vi "VHistory - Control Center.vi"(4 "value condition":T2 {"Range_Max" format="%<%H:%M:%S%2u>t"; "Range_Min" format="%<%H:%M:%S%2u>t"; "Delta" format="%<%H:%M:%S%2u>t"}, 6 "time conditions":cluster{"Step, ms":u32, "Gate, ms":u32}, 7 "VC Handle":T4=-1, 8 "error in":errorcluster, 9 "cmd (nop:default)":T3(ring), 10 "history length":i32, 11 "name_spec":string) -> (0 "error out":errorcluster, 2 "history info":T1 {"last time, sec" format="%<%H:%M:%S%2u\n%d/%m/%Y>T"; "value condition"."Range_Max" format="%<%H:%M:%S%2u>t"; "value condition"."Range_Min" format="%<%H:%M:%S%2u>t"; "value condition"."Delta" format="%<%H:%M:%S%2u>t"}, 3 "dup name_spec":string)   [LabVIEW 2021]
doc: "The VI is obsolete. It only exists to provide compatibility with VarMan 2.1. Use 'VHistory - History Controller.vi' instead of this VI.\n\n::: CalcExpress Toolkit :::\nCopyright (c) 2000-2026 Konstantin Shifershteyn. All rights reserved."
uses:
  cetypes.llb/VarMan Variable Context Handle.ctl
panel:
  # "THIS VI IS OBSOLETE"
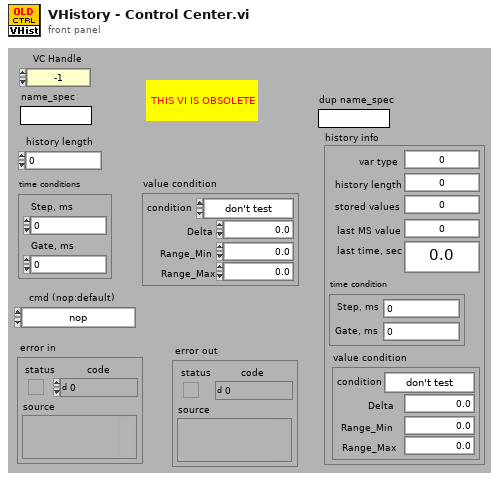
[diagram p1: front panel]
types:
  T1 = cluster{"var type":u32, "history length":i32, "stored values":i32, "last MS value":u32, "last time, sec":dbl, "time condition":cluster{"Step, ms":u32, "Gate, ms":u32}, "value condition":cluster{"condition":enum32{"don't test", "changed", "abs deviation", "rel deviation", "out of range", "within range"}, "Delta":dbl, "Range_Min":dbl, "Range_Max":dbl}}
  T2 = cluster{"condition":enum32{"don't test", "changed", "abs deviation", "rel deviation", "out of range", "within range"}, "Delta":dbl, "Range_Min":dbl, "Range_Max":dbl}
  T3 = enum32{"nop", "create", "destroy", "reset", "get info", "config"}
  T4 = typedef "VarMan Variable Context Handle.ctl" = i32
  T5 = typedef "VarMan History Info.ctl" = cluster{"var type":u32, "history length":u32, "stored values":u32, "update cnt":u32, "last update ms":u32, "newest timestamp":dbl, "oldest timestamp":dbl, "NewVals mode":cluster{"NewVals cnt":u32, "last read time":dbl, "last read ms":u32}, "time condition":cluster{"Step, ms":u32, "Gate, ms":u32}, "value condition":cluster{"condition":enum32{"don't test", "changed", "abs deviation", "rel deviation", "out of range", "within range"}, "Delta":dbl, "Range_Min":dbl, "Range_Max":dbl}}
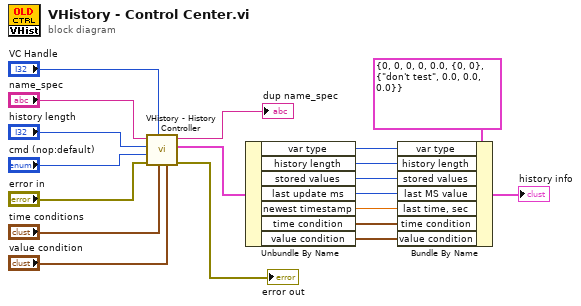
[diagram p0: block diagram]
diagram:
  n1 = call "VHistory - History Controller.vi"("value condition"="value condition", "time conditions"="time conditions", "VC Handle"="VC Handle", "error in"="error in", "cmd (nop:default)"="cmd (nop:default)", "history length"="history length", "name_spec"="name_spec") -> ("error out"=→"error out":errorcluster, "history info"=w10:T5, "dup name_spec"=→"dup name_spec":string)  [unwired: 1 in, 1 out]
  n2 = Unbundle By Name(w10) -> ("var type"=w9:u32, "history length"=w8:u32, "stored values"=w7:u32, "last update ms"=w6:u32, "newest timestamp"=w5:dbl, "time condition"=w4:cluster{"Step, ms":u32, "Gate, ms":u32}, "value condition"=w3:T2)
  n3 = Bundle By Name(cluster=T1 {"var type"=0, "history length"=0, "stored values"=0, "last MS value"=0, "last time, sec"=0.0, "time condition"={"Step, ms"=0, "Gate, ms"=0}, "value condition"={"condition"=enum."don't test", "Delta"=0.0, "Range_Min"=0.0, "Range_Max"=0.0}} ("history info"), "var type"=w9, "history length"=w8, "stored values"=w7, "last MS value"=w6, "last time, sec"=w5, "time condition"=w4, "value condition"=w3) -> (→"history info":T1)
